vi "Shared_DCPower_Start.vi"(10 "Pins":tag[](array[tag]), 11 "Semiconductor Module Context":T1) -> (0 "error Out":errorcluster)   [LabVIEW 2023, in "Shared.lvlib"]
doc: "Start supplying Voltage on the System Power Supply for Relay control"
uses:
  Shared.lvlib
  <vilib>/NI_TestStand_SemiconductorModule/NI_TestStand_Semiconductor_Module.lvlibp/PinMap/General/SemiconductorModuleContext.ctl
  <vilib>/NI_TestStand_SemiconductorModule/NI_TestStand_Semiconductor_Module.lvlibp/PinMap/DC Power/PinsToNIDCPowerSessions.vi
  <vilib>/NI_TestStand_SemiconductorModule/NI_TestStand_Semiconductor_Module.lvlibp
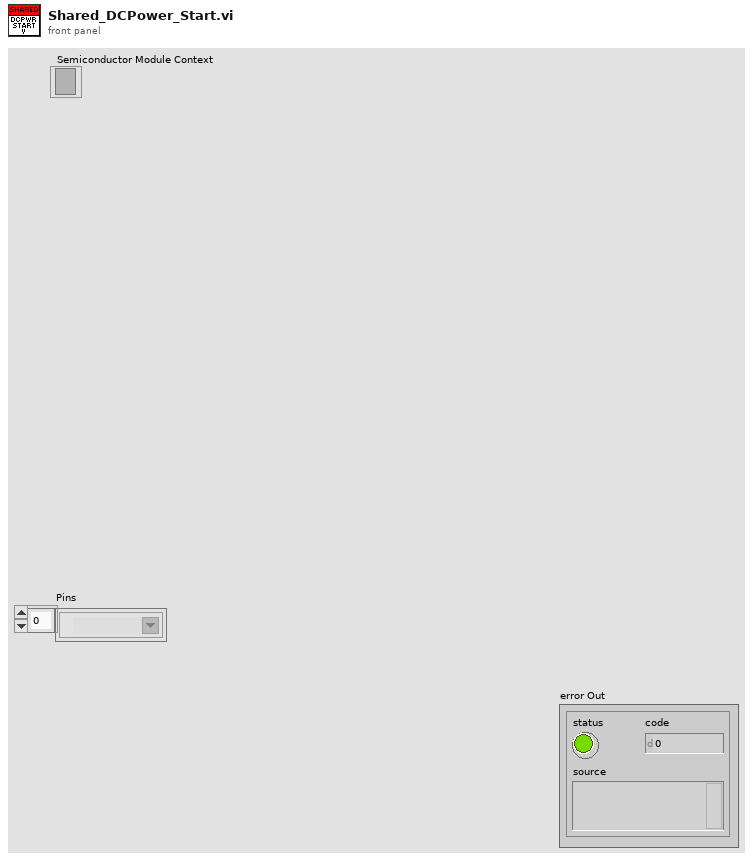
[diagram p1: front panel]
types:
  T1 = typedef "NI_TestStand_Semiconductor_Module.lvlibp/SemiconductorModuleContext.ctl" = refnum<k7>
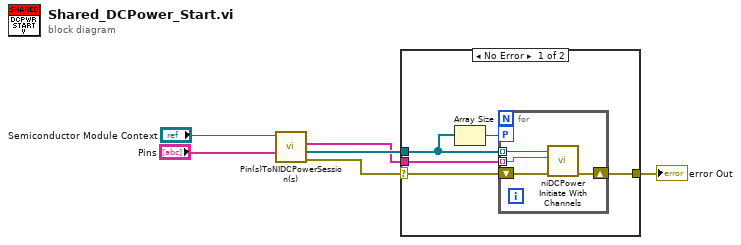
[diagram p0: block diagram]
diagram:
  n1 = call-poly <vilib>:"Pin(s)ToNIDCPowerSession(s).vi"("Pins"="Pins", "Semiconductor Module Context"="Semiconductor Module Context") -> ("error out"=w5:errorcluster, "Instrument Sessions"=w4:refnum<k15>[], "Channel Strings"=w3:string[])  [unwired: 5 in, 2 out]
  n2 = case shown="No Error" w5 {
    selector: w5 -> [w7 w16]
    tunnel: w4 -> [w10 _]
    tunnel: w3 -> [w9 _]
    tunnel: [w8 w16] -> w2
    frame No Error {
      n3 = Array Size(array=w10) -> (size(s)=w11:i32)
      n4 = for {
        tunnel: w10 -> [w15] mode=indexing
        workers-P: w11 -> [_]
        tunnel: w9 -> [w14] mode=indexing
        shift-right: [w13] -> w8
        shift-left: w7 -> [w12]
        n5 = call <instrlib>:"niDCPower Initiate With Channels.vi"("error in (no error)"=w12, "channel name"=w14, "instrument handle"=w15) -> ("error out"=w13:errorcluster)  [unwired: 7 in, 1 out]
      }
    }
    frame Error {
    }
  }
  "error Out" <- w2
